vi "GenerateAlotOfSignals.vi"(9 "Time":timestamp, 11 "Channels":i32) -> (3 "DAQ":T1 {"data" format="%.2f"; "status" format="%08x"})   [LabVIEW 2020, in "Sgraph_lib_V1.lvlib"]
doc: "Generate some DAQ data (should later be the benchmark) to test the data historian."
uses:
  HISW/controls/typedef_PAQsample.ctl
  Builds/Sgraph_lib_V1.lvlib
  <vilib>/ptbypt/NI_PtbyPt.lvlib
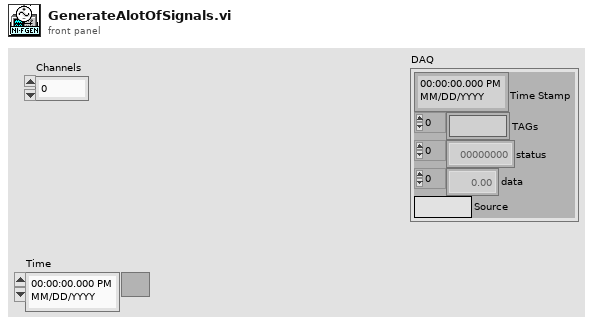
[diagram p1: front panel]
types:
  T1 = typedef "typedef_PAQsample.ctl" = cluster{"Time Stamp":timestamp, "TAGs":string[], "status":u32[], "data":dbl[], "Source":string}
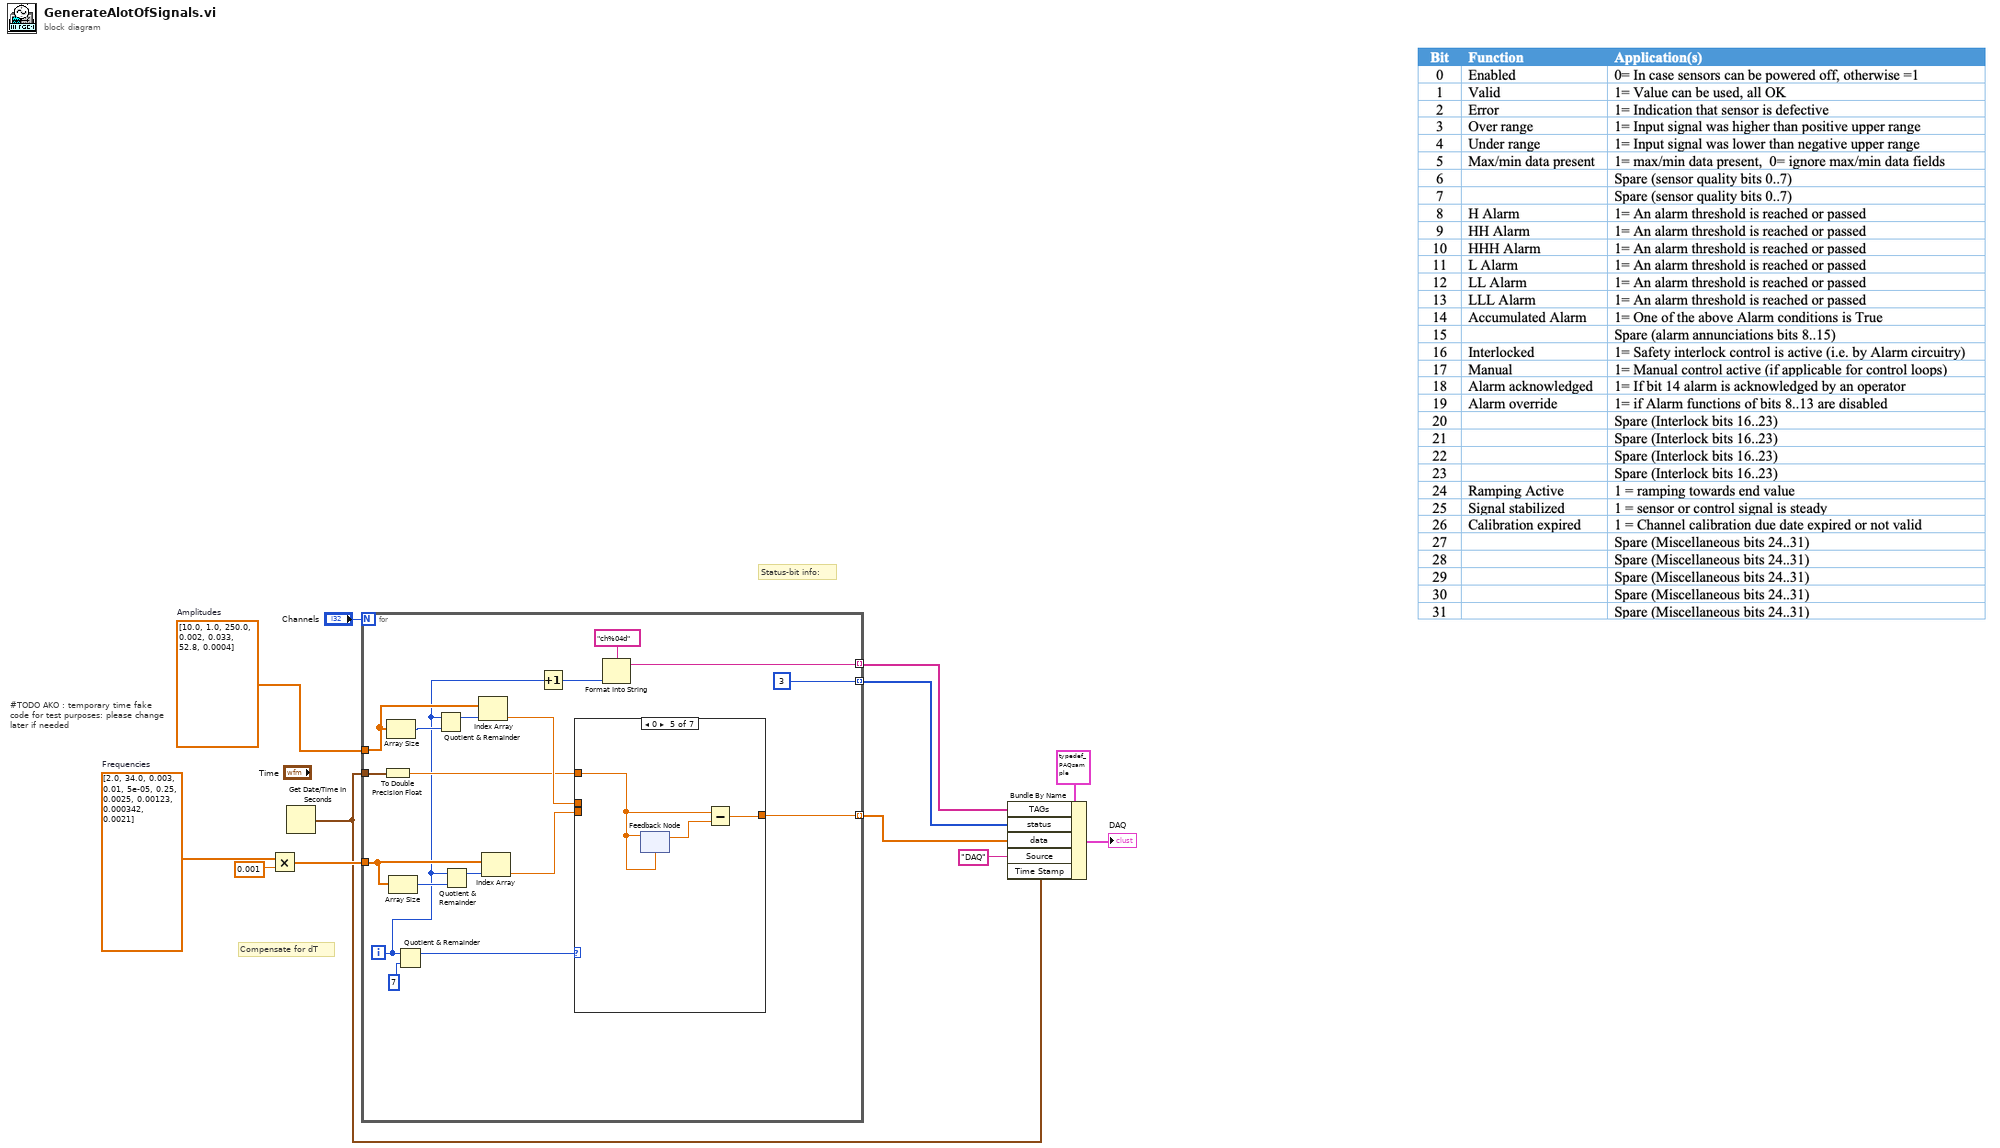
[diagram p0: block diagram]
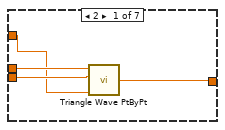
[diagram p2: hidden frame]
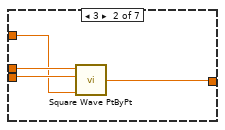
[diagram p3: hidden frame]
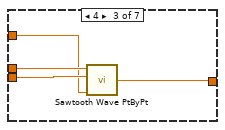
[diagram p4: hidden frame]
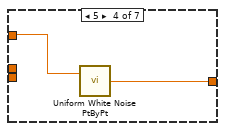
[diagram p5: hidden frame]
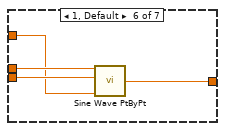
[diagram p6: hidden frame]
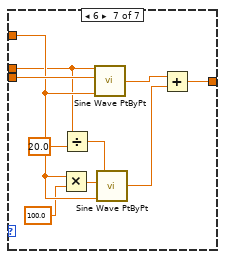
[diagram p7: hidden frame]
diagram:
  w12 = dbl[] [10.0, 1.0, 250.0, 0.002, 0.033, 52.8, 0.0004]  # Amplitudes
  w5 = dbl[] [2.0, 34.0, 0.003, 0.01, 5e-05, 0.25, 0.0025, 0.00123, 0.000342, 0.0021]  # Frequencies
  # "#TODO AKO : temporary time fake\ncode for test purposes: please change\nlater if needed"
  # "Compensate for dT"
  # "Status-bit info:"
  n1 = Multiply(x=w5, y=0.001) -> (x*y=w4:dbl[])
  n2 = Get Date/Time In Seconds() -> (seconds since 1Jan1904=w1:timestamp)
  n3 = for {
    N: "Channels" -> [_]
    tunnel: w12 -> [w25]
    tunnel: w4 -> [w27]
    tunnel: w1 -> [w20]
    tunnel: [w13] -> w8 mode=indexing
    tunnel: [w15] -> w10 mode=indexing
    tunnel: [u32 3] -> w9 mode=indexing
    i -> [w18]
    n4 = To Double Precision Float(number=w20) -> (double precision float=w19:dbl)
    n5 = Array Size(array=w25) -> (size(s)=w28:i32)
    n6 = Array Size(array=w27) -> (size(s)=w29:i32)
    n7 = Quotient & Remainder(x=w18, y=7) -> (x-y*floor(x/y)=w23:i32)  [unwired: 1 out]
    n8 = Quotient & Remainder(x=w18, y=w28) -> (x-y*floor(x/y)=w24:i32)  [unwired: 1 out]
    n9 = Quotient & Remainder(x=w18, y=w29) -> (x-y*floor(x/y)=w26:i32)  [unwired: 1 out]
    n10 = Index Array(array=w25, index=w24) -> (element=w22:dbl)
    n11 = Index Array(array=w27, index=w26) -> (element=w21:dbl)
    n12 = Increment(x=w18) -> (x+1=w17:i32)
    n13 = case shown="0" w23 {
      tunnel: w22 -> [w34 w38 w42 _ _ w51 w57]
      tunnel: w21 -> [w33 w36 w41 _ _ w50 w61]
      tunnel: w19 -> [w32 w35 w40 w44 w45 w49 w59]
      tunnel: [w31 w37 w39 w43 w46 w48 w52] -> w13
      frame 2 {
        n14 = call <vilib>:"Triangle Wave PtByPt.vi"("time"=w32, "frequency"=w33, "amplitude"=w34) -> ("triangle wave"=w31:dbl)  [unwired: 1 in]
      }
      frame 3 {
        n15 = call <vilib>:"Square Wave PtByPt.vi"("amplitude"=w38, "frequency"=w36, "time"=w35) -> ("square wave"=w37:dbl)  [unwired: 2 in]
      }
      frame 4 {
        n16 = call <vilib>:"Sawtooth Wave PtByPt.vi"("time"=w40, "frequency"=w41, "amplitude"=w42) -> ("sawtooth wave"=w39:dbl)  [unwired: 1 in]
      }
      frame 5 {
        n17 = call <vilib>:"Uniform White Noise PtByPt.vi"("amplitude"=w44) -> ("uniform white noise"=w43:dbl)  [unwired: 2 in]
      }
      frame 0 {
        n18 = feedback #1(w45) -> (w47:dbl)
        n19 = feedback-in #1(w45) -> ()
        n20 = Subtract(x=w45, y=w47) -> (x-y=w46:dbl)
      }
      frame 1, Default {
        n21 = call <vilib>:"Sine Wave PtByPt.vi"("time"=w49, "frequency"=w50, "amplitude"=w51) -> ("sine wave"=w48:dbl)  [unwired: 1 in]
      }
      frame 6 {
        n22 = Multiply(x=w59, y=100.0) -> (x*y=w60:dbl)
        n23 = Divide(x=w57, y=20.0) -> (x/y=w55:dbl)
        n24 = call <vilib>:"Sine Wave PtByPt.vi"("time"=w59, "frequency"=w61, "amplitude"=w57) -> ("sine wave"=w53:dbl)  [unwired: 1 in]
        n25 = call <vilib>:"Sine Wave PtByPt.vi"("time"=w59, "frequency"=w60, "amplitude"=w55) -> ("sine wave"=w54:dbl)  [unwired: 1 in]
        n26 = Add(x=w53, y=w54) -> (x+y=w52:dbl)
      }
    }
    n27 = Format Into String(format string="ch%04d", w17) -> (resulting string=w15:string)  [unwired: 2 in, 1 out]
  }
  n28 = Bundle By Name(cluster=T1 {"Time Stamp"=timestamp(0 s since 1904-01-01), "TAGs"=[], "status"=[], "data"=[], "Source"=""} ("PAQsample"), "TAGs"=w10, "status"=w9, "data"=w8, "Source"="DAQ", "Time Stamp"=w1) -> (→"DAQ":T1)
